vi "Refresh All Nodes.vi"(8 "error in (no error)":errorcluster, 10 "summary":T1[](array[typedef])) -> (0 "error out":errorcluster)   [LabVIEW 2013, in "Standard Editor.lvlib"]
uses:
  Standard Editor.lvlib
  <vilib>/NI/Configuration Framework/Node/Summary.ctl
  Configuration Editor/Classes/Module editor node/module editor node.lvclass
  Configuration Editor/Classes/Engine Parent/read engine configuration.vi
  Configuration Editor/Classes/Engine Parent/write engine configuration.vi
  <vilib>/NI/Module Execution Interface/Engine Configuration/engine configuration.lvclass
  <vilib>/NI/Configuration Framework/Node/NISE_CEF_Node.lvclass
  Configuration Editor/Classes/Engine Parent/Engine Parent Editor Node.lvclass
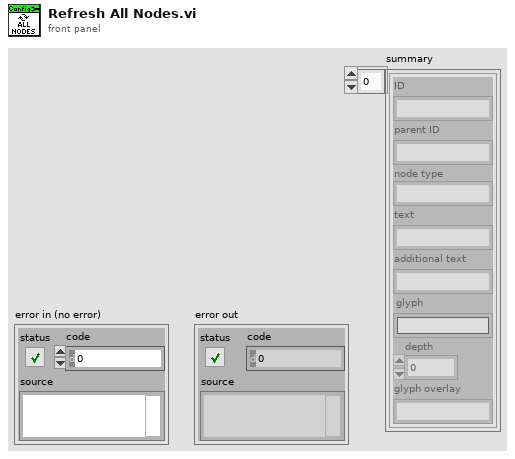
[diagram p1: front panel]
types:
  T1 = typedef "NISE_CEF_Node.lvclass/Summary.ctl" = cluster{"ID":string, "parent ID":string, "node type":string, "text":string, "additional text":string, "glyph":string, "depth":i32, "glyph overlay":string}
  T2 = typedef "NISE_CEF_Node.lvclass/NodeRef.ctl" = refnum<data-value>
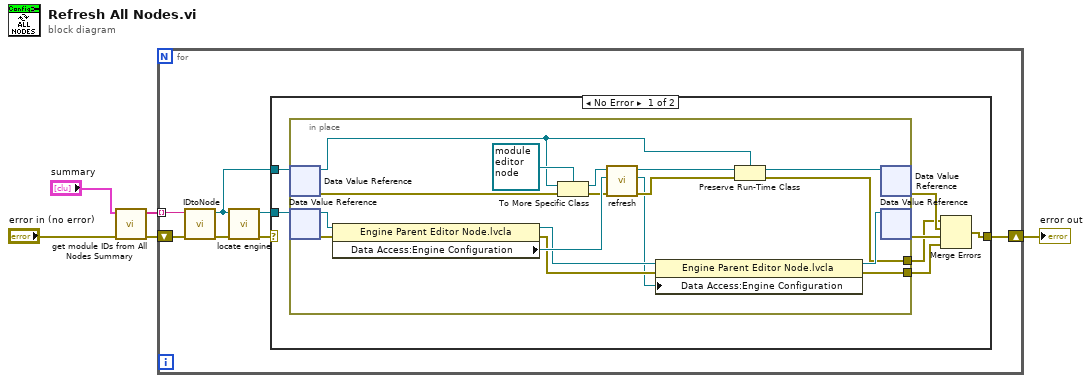
[diagram p0: block diagram]
diagram:
  n1 = call "get module IDs from All Nodes Summary.vi"("error in (no error)"="error in (no error)", "summary"="summary") -> ("error out"=w1:errorcluster, "module IDs"=w3:string[])  [unwired: 8 in]
  n2 = for {
    tunnel: w3 -> [w12] mode=indexing
    shift-right: [w6] -> w5
    shift-left: w1 -> [w11]
    n3 = call <vilib>:"IDtoNode.vi"("error in"=w11, "ID"=w12) -> ("error out"=w10:errorcluster, "node ref"=w8:T2)  [unwired: 7 in, 1 out]
    n4 = call "locate engine.vi"("error in"=w10, "component"=w8) -> ("error out"=w7:errorcluster, "engine"=w9:refnum<data-value>)  [unwired: 8 in]
    n5 = case shown="No Error" w7 {
      selector: w7 -> [_ w37]
      tunnel: w9 -> [w19 _]
      tunnel: w8 -> [w18 _]
      tunnel: [w13 w37] -> w6
      frame No Error {
        n6 = in-place {
          in-place-border: [w27] -> w17
          in-place-border: [w22] -> w14
          n7 = in-place-dvr #1(w18) -> (w25:refnum<class "NISE_CEF_Node.lvclass">, w36:errorcluster)
          n8 = in-place-dvr #2(w19) -> (w34:refnum<class "Engine Parent Editor Node.lvclass">, w29:errorcluster)
          n9 = property class="Engine Parent Editor Node.lvcla"(reference=w34, error in=w29) -> (reference out=w31:refnum<class "Engine Parent Editor Node.lvclass">, error out=w30:errorcluster, "Data Access:Engine Configuration"=w32:refnum<class "engine configuration.lvclass">)
          n10 = To More Specific Class(target class=refnum<class "module editor node.lvclass"> refnum ("Tag Editor Core:module editor node"), reference=w25, error in=w36) -> (specific class reference=w33:refnum<class "module editor node.lvclass">, error out=w21:errorcluster)
          n11 = call-dynamic "refresh.vi"("error in (no error)"=w21, "Engine Configuration In"=w32, "Module Editor Node In"=w33) -> ("error out"=w23:errorcluster, "Engine Configuration Out"=w20:refnum<class "engine configuration.lvclass">, "Module Editor Node Out"=w26:refnum<class "module editor node.lvclass">)  [unwired: 6 in]
          n12 = property class="Engine Parent Editor Node.lvcla"(reference=w31, error in=w30, "Data Access:Engine Configuration"=w20) -> (reference out=w28:refnum<class "Engine Parent Editor Node.lvclass">, error out=w27:errorcluster)
          n13 = Preserve Run-Time Class(object in=w26, error in=w23, 2:w25) -> (object out=w24:refnum<class "NISE_CEF_Node.lvclass">, error out=w22:errorcluster)
          n14 = in-place-dvr #1(w24) -> (w15:errorcluster)  [unwired: 1 out]
          n15 = in-place-dvr #2(w28) -> (w16:errorcluster)  [unwired: 1 out]
        }
        n16 = Merge Errors(w14, w15, w16, w17) -> (w13:errorcluster)
      }
      frame Error {
      }
    }
  }
  "error out" <- w5
